vi "ziExample-Module-DataStreaming.vi"() -> ()   [LabVIEW 2009]
doc: "Control a Zurich instrument device via the LabOne Labview API. \nRequirements: Zurich Instruments MFLI, HF2 or UHFLI \nThis example shows how to start a DAQ trigger module and retrieve the Data.\n\n© Zurich Instruments AG, www.zhinst.com"
uses:
  <instrlib>/Zurich Instruments LabOne/Public/Modules/ziTypeModEnum.ctl
  <instrlib>/Zurich Instruments LabOne/Public/Modules/ziModSetValueDouble.vi
  <instrlib>/Zurich Instruments LabOne/Public/Modules/ziModGetDoubleData.vi
  <instrlib>/Zurich Instruments LabOne/Public/Modules/ziModGetUnsignedIntegerData.vi
  <instrlib>/Zurich Instruments LabOne/Public/Utility/ziTicksToS_vector.vi
  <instrlib>/Zurich Instruments LabOne/Zurich Instruments LabOne.lvlib
  <instrlib>/Zurich Instruments LabOne/Private/ziLV64.dll
panel:
  out "Finished?":bool
  out "Progress (%)":dbl
  out "Actual duration":dbl=1.0 caption="Actual  duration" format="%_5g"
  out "Selected Device":string
  in  "subscribe":string[](array[string])=["demods/0/sample.x", "demods/0/sample.y", "demods/0/sample.r"] caption="Subscribe Paths"
  out "XY Graph":cluster{"Timestamp(s)":dbl[], "Value":dbl[]}[](graph)
  in  "Stop":bool
  in  "duration":dbl=1.0 caption="Duration" format="%#_8g"
  out "Error Out":errorcluster
  in  "Address":string="DEV"
  # "For endless acquisition, set the duration to 0 and use the STOP button to end the capture"
  # "ziExample-Module-Data_Streaming.vi\nRequirements: \n- Any Zurich Instruments Lock-In with at least 1 demodulator \nsee block diagram for VI description"
  # "Tested Instruments:\n- HF2LI\n- UHFLI\n- MFLI\n- SHFLI\n- GHFLI\n- VHFLI"
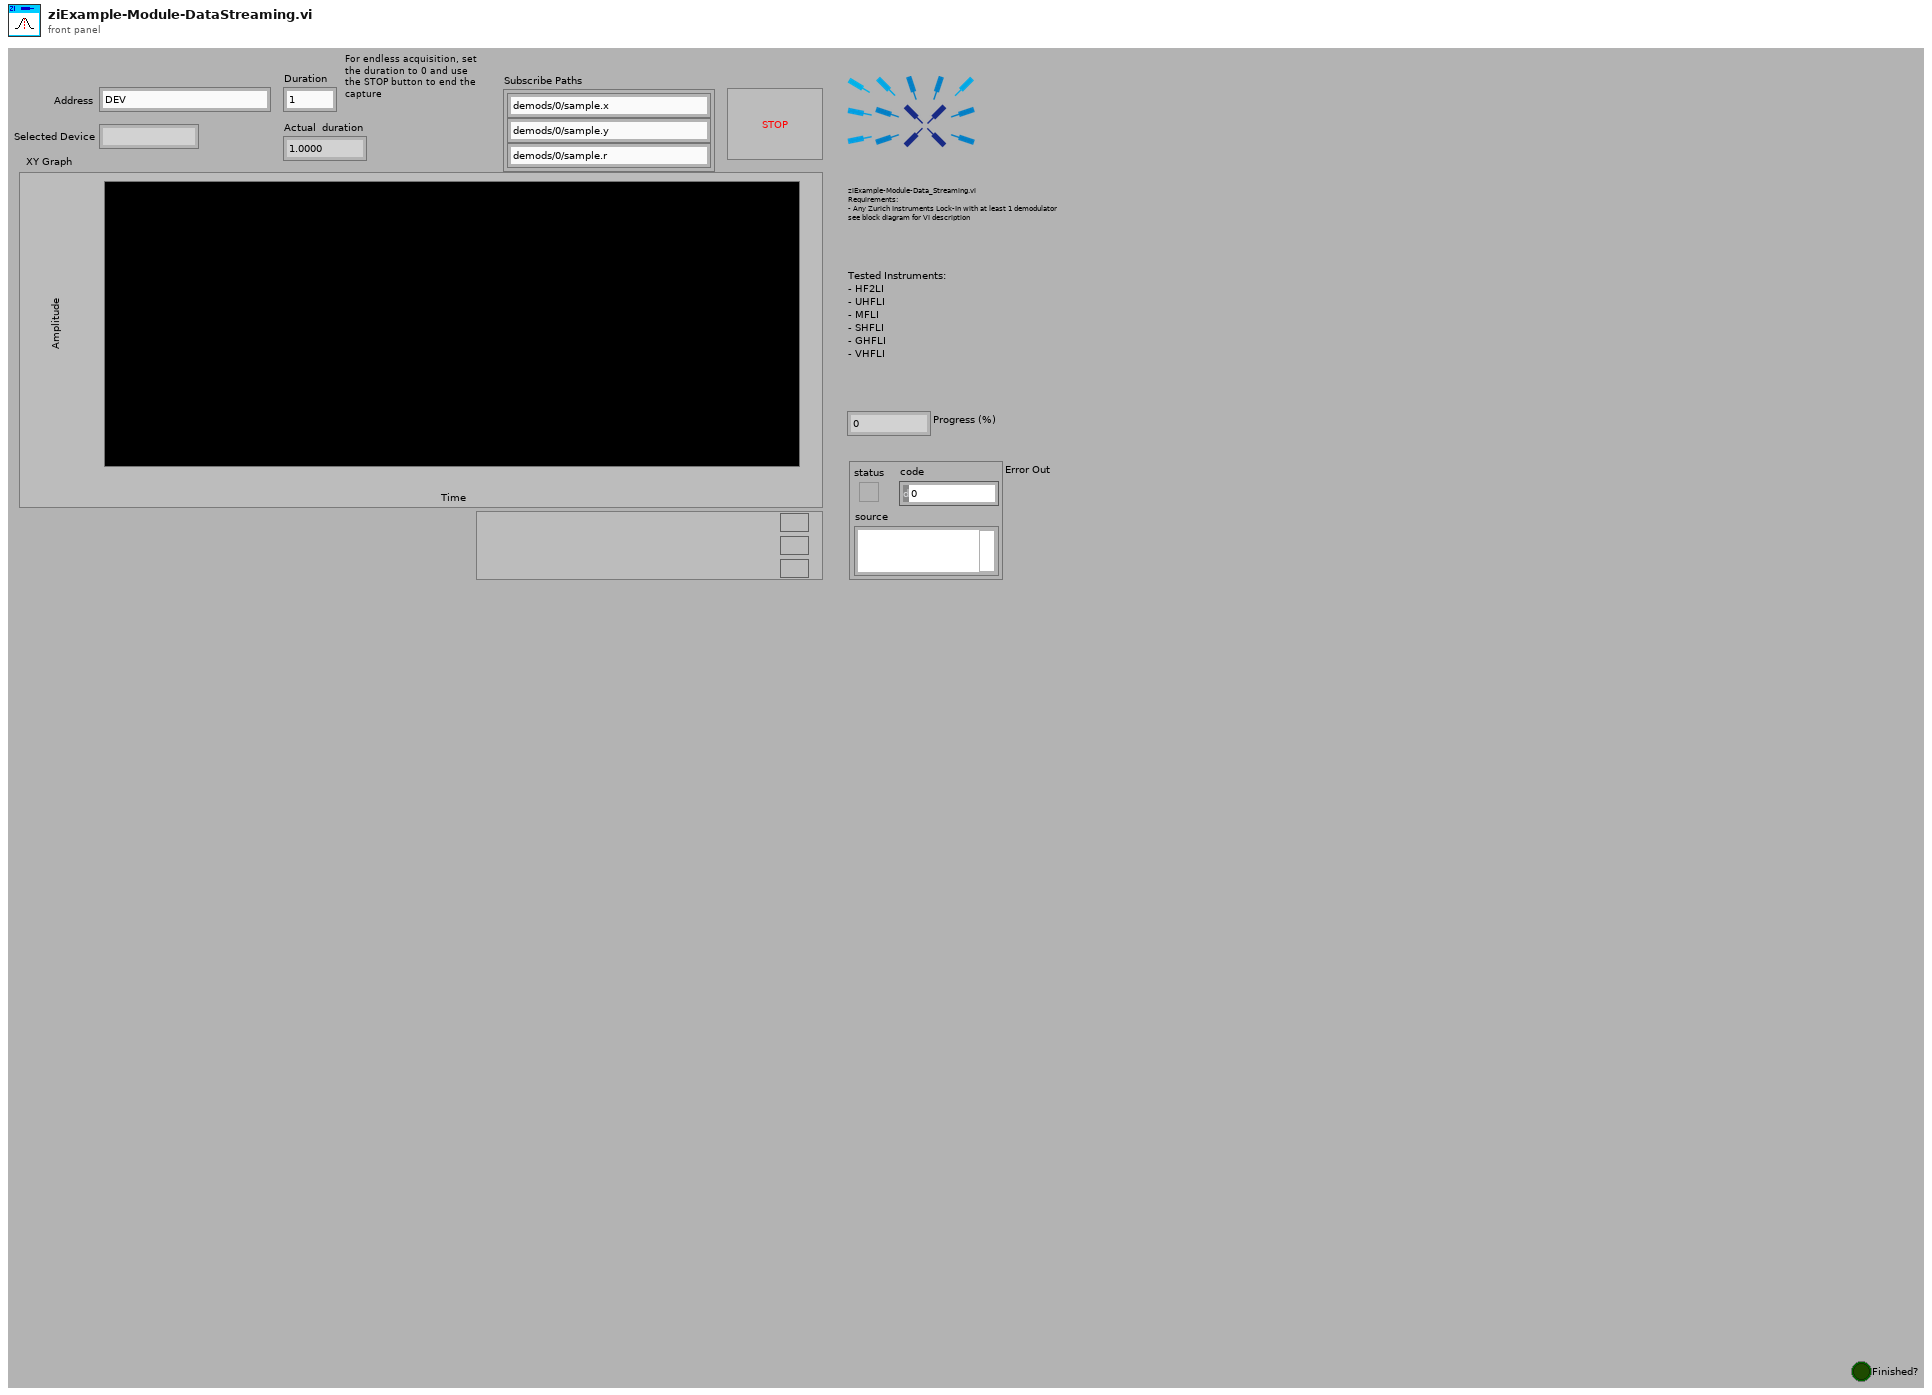
[diagram p1: front panel]
types:
  T1 = typedef "Zurich Instruments LabOne.lvlib/ziTypeModEnum.ctl" = u16
  T2 = typedef "Zurich Instruments LabOne.lvlib/ziTypeHandle.ctl" = cluster{"handleValid":bool, "Conn":u64, "Path Prefix":string, "Handle":u64, "Connected":bool, "Clockbase(s)":dbl}
  T3 = typedef "Zurich Instruments LabOne.lvlib/ziTypeModHandle.ctl" = cluster{"handleValid":bool, "Conn":u64, "ModHandle":u64, "moduleID":string, "Path Prefix":string}
  T4 = typedef "Zurich Instruments LabOne.lvlib/ziTypeModResults.ctl" = cluster{"PathArray":string[], "ValueType":T5, "NoOfResults":u64, "ziGenericHeader":T6[]}
  T5 = typedef "Zurich Instruments LabOne.lvlib/ziTypePollType.ctl" = enum16{"NONE", "DOUBLE_DATA", "INTEGER_DATA", "DEMOD_SAMPLE", "SCOPE_WAVE_HF2", "AUXIN_SAMPLE", "DIO_SAMPLE", "BYTE_ARRAY", "PWA_WAVE", "9", "10", "11", "12", "13", "14", "15", "TREE_CHANGE_DEPRI", "17", "ERROR", "19", "20", "21", "22", "23", "24", "25", "26", "27", "28", "29", "30", "31", "DOUBLE_DATA_TS", "INTEGER_DATA_TS", "34", "SCOPE_WAVE", "SCOPE_WAVE_EX", "37", "BYTE_ARRAY_TS", "39", "40", "41", "42", "43", "44", "45", "CNT_DATA", "47", "TREE_CHANGE", "49", "50", "51", "52", "53", "54", "55", "56", "57", "58", "59", "60", "61", "62", "63", "SWEEPER_DATA", "SPECTRUM_DATA", "ADVISOR_DATA", "VECTOR_DATA", "IMP_DATA", "SHF_GENERATOR_WAVEFORM_DATA", "SHF_RESULT_LOGGER_DATA", "SHF_SCOPE_DATA", "DEMOD_VECTOR", "73", "PID_VECTOR", "UNSIGNED_INTEGER_DATA"}
  T6 = typedef "Zurich Instruments LabOne.lvlib/ziTypeModGenericHeader.ctl" = cluster{"HeaderType":enum8{"HEADER_TYPE_NONE", "HEADER_TYPE_SWTRIGGER", "HEADER_TYPE_SWEEPER"}, "SampleFormat":u8, "SystemTime":timestamp, "CreatedTimeStamp":u64, "ChangedTimeStamp":u64, "Flags":u32, "ChunkSizeBytes":u64, "Name":string, "Status":u32, "GroupIndex":u32, "Color":u32, "ActiveRow":u32, "TriggerNumber":u64, "GridRows":u32, "GridCols":u32, "GridMode":u32, "GridOperation":u32, "GridDirection":u32, "GridRepetitions":u32, "GridColDelta":dbl, "GridColOffset":dbl, "GridRowDelta":dbl, "GridRowOffset":dbl, "Bandwidth":dbl, "Center":dbl, "Nenbw":dbl}
  T7 = typedef "Zurich Instruments LabOne.lvlib/ziTypeDoubleDataTS.ctl" = cluster{"Timestamp (ticks)":u64[], "Value":dbl[]}
  T8 = typedef "Zurich Instruments LabOne.lvlib/ziTypeUnsignedIntegerData.ctl" = cluster{"Value":u64[]}
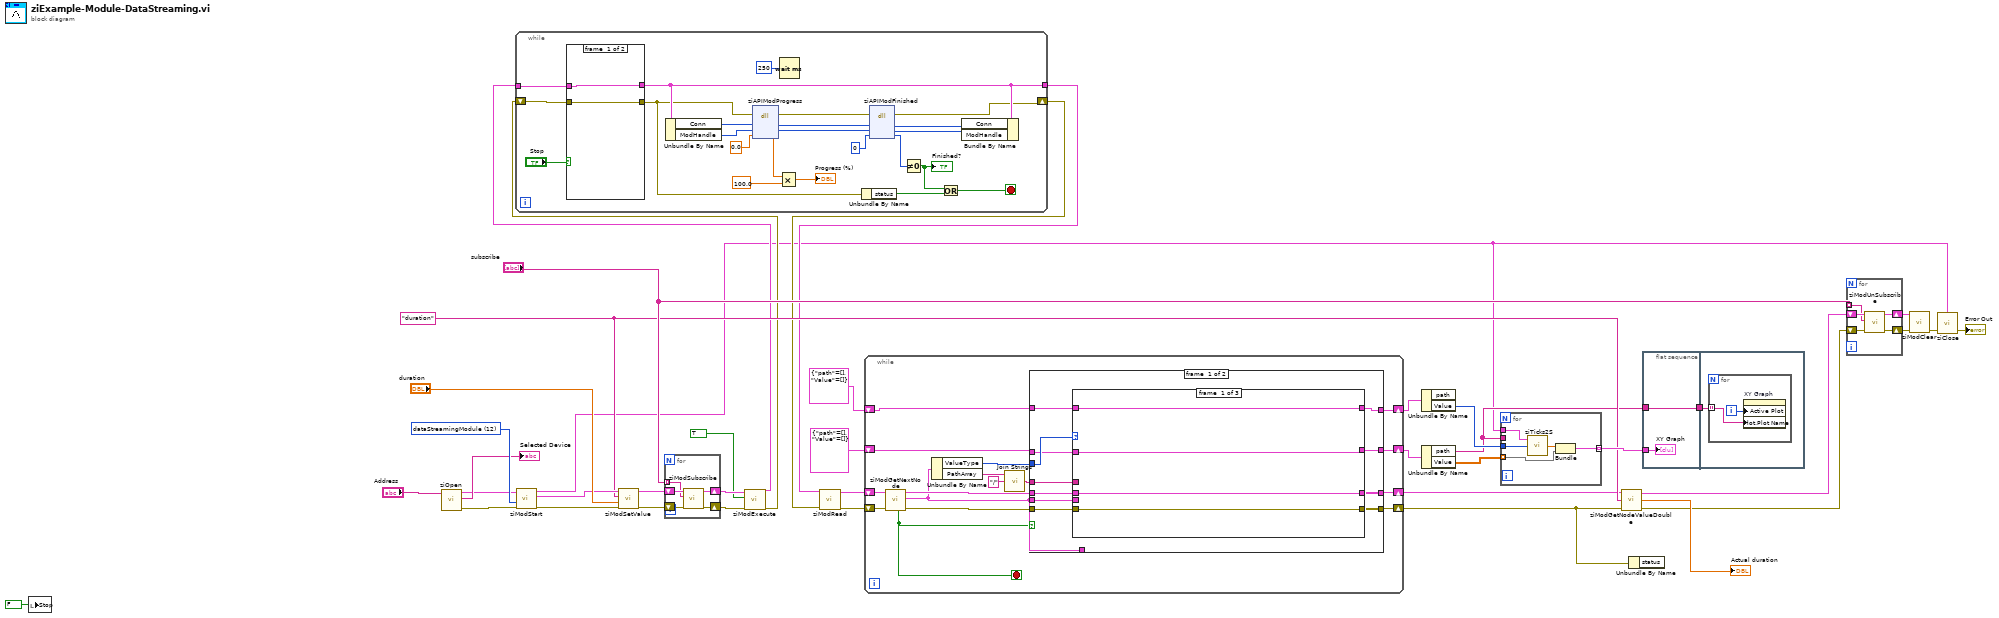
[diagram p0: block diagram]
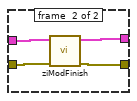
[diagram p2: hidden frame]
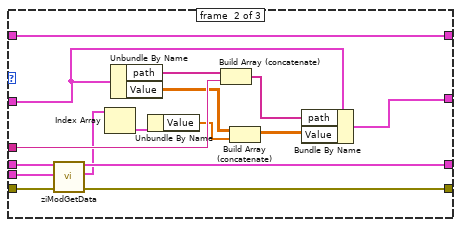
[diagram p3: hidden frame]
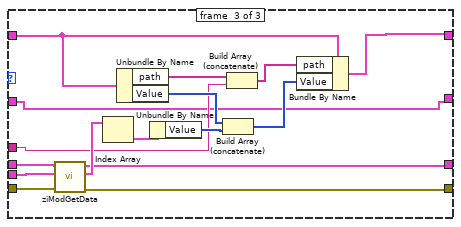
[diagram p4: hidden frame]
diagram:
  w14 = "duration"
  w32 = T1 12 items=["sweep", "scopeModule", "dataAcquisitionModule", "pidAdvisor", "awgModule", "impedanceModule", "multiDeviceSyncModule", "zoomFFT", "trigger", "deviceSettings", "record", "precompensationAdvisor", "dataStreamingModule"] ("module Id")
  n1 = local write "Stop"(FALSE ("run")) -> ()
  n2 = call <instrlib>:"ziOpen.vi"("Address"="Address") -> ("HandleOut"=w1:T2, "Selected Device"=→"Selected Device":string, "Error Out"=w37:errorcluster)  [unwired: 5 in]
  n3 = call <instrlib>:"ziModStart.vi"("Error In"=w37, "module Id"=w32, "Handle In"=w1) -> ("Error Out"=w27:errorcluster, "ModHandle Out"=w26:T3, "Handle Out"=w2:T2)  [unwired: 6 in]
  n4 = call-poly <instrlib>:"ziModSetValue.vi"("Error In"=w27, "Value"="duration", "Path"=w14, "ModHandle In"=w26) -> ("Error Out"=w33:errorcluster, "ModHandle Out"=w34:T3)  [unwired: 6 in]
  n5 = for {
    tunnel: "subscribe" -> [w42] mode=indexing
    shift-right: [w46] -> w36
    shift-left: w34 -> [w44]
    shift-right: [w45] -> w35
    shift-left: w33 -> [w43]
    n6 = call <instrlib>:"ziModSubscribe.vi"("Error In"=w43, "Path"=w42, "ModHandle In"=w44) -> ("Error Out"=w45:errorcluster, "ModHandle Out"=w46:T3)  [unwired: 6 in]
  }
  n7 = call <instrlib>:"ziModExecute.vi"("Error In"=w35, "Modal (F)"=TRUE, "ziModHandle In"=w36) -> ("Error Out"=w10:errorcluster, "ziModHandle Out"=w7:T3)  [unwired: 6 in]
  n8 = while {
    shift-right: [w51] -> w3
    shift-left: w10 -> [w69]
    tunnel: w7 -> [w68]
    tunnel: [w52] -> w4
    stop <- w49 stop-if-true
    n9 = case shown="False" "Stop" {
      tunnel: w69 -> [w71 w75]
      tunnel: [w71 w72] -> w48
      tunnel: [w70 w73] -> w52
      tunnel: w68 -> [w70 w74]
      frame #0 {
      }
      frame #1 {
        n10 = call <instrlib>:"ziModFinish.vi"("Error In"=w75, "ziModHandle In"=w74) -> ("Error Out"=w72:errorcluster, "ziModHandle Out"=w73:T3)  [unwired: 7 in]
      }
    }
    n11 = Unbundle By Name(w52) -> ("Conn"=w63:u64, "ModHandle"=w64:u64)
    n12 = dll-call lib="C:/Program Files/National Instruments/LabVIEW 2009/instr.lib/Zurich Instruments LabOne/Private/ziLV*.*" fn="ziAPIModProgress"(error in=w48, "conn"=w63, "ModHandle"=w64, "Finished"=0.0) -> (error out=w59:errorcluster, "conn"=w58:u64, "ModHandle"=w53:u64, "Finished"=w61:dbl)  [unwired: 2 in, 2 out]
    n13 = Multiply(x=w61, y=100.0) -> (x*y=→"Progress (%)":dbl)
    n14 = Wait (ms)(milliseconds to wait=u32 250) -> ()  [unwired: 1 out]
    n15 = Unbundle By Name(w48) -> ("status"=w47:bool)
    n16 = dll-call lib="C:/Program Files/National Instruments/LabVIEW 2009/instr.lib/Zurich Instruments LabOne/Private/ziLV*.*" fn="ziAPIModFinished"(error in=w59, "conn"=w58, "ModHandle"=w53, "Finished"=i64 0) -> (error out=w51:errorcluster, "conn"=w65:u64, "ModHandle"=w66:u64, "Finished"=w54:i64)  [unwired: 2 in, 2 out]
    n17 = Not Equal To 0?(x=w54) -> (x != 0?=w50:bool)
    "Finished?" <- w50
    n18 = Or(x=w50, y=w47) -> (x .or. y?=w49:bool)
    n19 = Bundle By Name(cluster=w52, "Conn"=w65, "ModHandle"=w66) -> ()  [unwired: 1 out]
  }
  n20 = call <instrlib>:"ziModRead.vi"("error in"=w3, "ziModHandle In"=w4) -> ("error out"=w9:errorcluster, "ziModHandle Out"=w8:T3)  [unwired: 8 in]
  n21 = while {
    shift-right: [w86] -> w6
    shift-left: w8 -> [w90]
    shift-right: [w87] -> w5
    shift-left: w9 -> [w91]
    shift-right: [w77] -> w18
    shift-left: cluster{"path":string[], "Value":u64[]} {"path"=[], "Value"=[]} ("DoubleSample") -> [w79]
    shift-right: [w78] -> w19
    shift-left: cluster{"path":string[], "Value":dbl[][]} {"path"=[], "Value"=[]} ("DoubleSample") -> [w82]
    stop <- w76 stop-if-true
    n22 = call <instrlib>:"ziModGetNextNode.vi"("Error In"=w91, "ModHandle In"=w90) -> ("Error Out"=w88:errorcluster, "ModResults"=w80:T4, "ModHandle Out"=w89:T3, "NoData"=w76:bool)  [unwired: 6 in]
    n23 = Unbundle By Name(w80) -> ("ValueType"=w83:T5, "PathArray"=w81:string[])
    n24 = call <vilib>:"Join Strings.vi"("Separator (,)"="/", "Strings In"=w81) -> ("String"=w84:string)  [unwired: 1 in]
    n25 = case shown="True" w76 {
      tunnel: w80 -> [_ _]
      tunnel: w89 -> [w95 w142]
      tunnel: w88 -> [w96 w141]
      tunnel: [w102 w141] -> w87
      tunnel: [w101 w142] -> w86
      tunnel: w84 -> [w98 _]
      tunnel: w83 -> [w100 _]
      tunnel: w82 -> [w99 w139]
      tunnel: w80 -> [w97 _]
      tunnel: w79 -> [w94 w140]
      tunnel: [w93 w139] -> w78
      tunnel: [w92 w140] -> w77
      frame #0 {
        n26 = case shown="\"DOUBLE_DATA\"" w100 {
          tunnel: w96 -> [w105 w119 w128]
          tunnel: [w105 w117 w126] -> w102
          tunnel: [w106 w115 w127] -> w101
          tunnel: w99 -> [w104 w109 w123]
          tunnel: w98 -> [_ w121 w131]
          tunnel: w97 -> [_ w118 w129]
          tunnel: w95 -> [w106 w116 w130]
          tunnel: w94 -> [w103 w108 w125]
          tunnel: [w104 w107 w123] -> w93
          tunnel: [w103 w108 w124] -> w92
          frame #0 {
          }
          frame #1 {
            n27 = call-poly <instrlib>:"ziModGetData.vi"("Error In"=w119, "ModResults"=w118, "ModHandle In"=w116) -> ("Error Out"=w117:errorcluster, "DoubleSample"=w114:T7[], "ModHandle Out"=w115:T3)  [unwired: 4 in, 2 out]
            n28 = Index Array(array=w114) -> (element=w113:T7)  [unwired: 1 in]
            n29 = Unbundle By Name(w109) -> ("path"=w122:string[], "Value"=w111:dbl[][])
            n30 = Unbundle By Name(w113) -> ("Value"=w110:dbl[])
            n31 = Build Array (concatenate)(w122, w121) -> (w120:string[])
            n32 = Build Array (concatenate)(w111, w110) -> (w112:dbl[][])
            n33 = Bundle By Name(cluster=w109, "path"=w120, "Value"=w112) -> (w107:cluster{"path":string[], "Value":dbl[][]})
          }
          frame #2 {
            n34 = call-poly <instrlib>:"ziModGetData.vi"("Error In"=w128, "ModResults"=w129, "ModHandle In"=w130) -> ("Error Out"=w126:errorcluster, "ModIUnsignedntegerData"=w137:T8[], "ModHandle Out"=w127:T3)  [unwired: 5 in, 1 out]
            n35 = Index Array(array=w137) -> (element=w136:T8)  [unwired: 1 in]
            n36 = Unbundle By Name(w125) -> ("path"=w132:string[], "Value"=w134:u64[])
            n37 = Unbundle By Name(w136) -> ("Value"=w138:u64[])
            n38 = Build Array (concatenate)(w134, w138) -> (w135:u64[])
            n39 = Build Array (concatenate)(w132, w131) -> (w133:string[])
            n40 = Bundle By Name(cluster=w125, "path"=w133, "Value"=w135) -> (w124:cluster{"path":string[], "Value":u64[]})
          }
        }
      }
      frame #1 {
      }
    }
  }
  n41 = Unbundle By Name(w18) -> ("Value"=w20:u64[])  [unwired: 1 out]
  n42 = Unbundle By Name(w19) -> ("path"=w13:string[], "Value"=w12:dbl[][])
  n43 = for {
    tunnel: w20 -> [w145]
    tunnel: w12 -> [w147] mode=indexing
    tunnel: [w144] -> w22 mode=indexing
    tunnel: w13 -> [_]
    tunnel: w2 -> [w143]
    n44 = call-poly <instrlib>:"ziTicks2S.vi"("Timestamp (ticks)"=w145, "Handle In"=w143) -> ("Timestamp(s)"=w146:dbl[])  [unwired: 1 in, 2 out]
    n45 = Bundle("Timestamp(s)"=w146, "Value"=w147) -> (w144:cluster{"Timestamp(s)":dbl[], "Value":dbl[]})  [unwired: 1 in]
  }
  n46 = call <instrlib>:"ziModGetNodeValueDouble.vi"("ModHandle In"=w6, "Path"=w14, "error in"=w5) -> ("ModHandle Out"=w15:T3, "Value"=→"Actual duration":dbl, "error out"=w16:errorcluster)  [unwired: 10 in]
  n47 = Unbundle By Name(w5) -> ()  [unwired: 1 out]
  n48 = flat-sequence {
    tunnel: w22 -> [w149]
    tunnel: [w148] -> w24
    tunnel: w13 -> [w148]
    tunnel: w24 -> [w150]
    frame #0 {
      "XY Graph" <- w149
    }
    frame #1 {
      n49 = for {
        tunnel: w150 -> [w152] mode=indexing
        i -> [w151]
        n50 = property on="XY Graph" class="XYGraph (strict)"("Active Plot"=w151, "Plot.Plot Name"=w152) -> ()  [unwired: 2 in, 2 out]
      }
    }
  }
  n51 = for {
    tunnel: "subscribe" -> [w153] mode=indexing
    shift-right: [w156] -> w39
    shift-left: w15 -> [w154]
    shift-right: [w157] -> w40
    shift-left: w16 -> [w155]
    n52 = call <instrlib>:"ziModUnSubscribe.vi"("Error In"=w155, "Path (\"/\")"=w153, "ModHandle In"=w154) -> ("Error Out"=w157:errorcluster, "ModHandle Out"=w156:T3)  [unwired: 7 in]
  }
  n53 = call <instrlib>:"ziModClear.vi"("Error In"=w40, "ziModHandle In"=w39) -> ("Error Out"=w31:errorcluster)  [unwired: 7 in, 1 out]
  n54 = call <instrlib>:"ziClose.vi"("Error In"=w31, "Handle In"=w2) -> ("Error Out"=→"Error Out":errorcluster)  [unwired: 2 in, 1 out]
